vi "SMTP Email Send Message End.vi"(4 "error in (no error)":errorcluster caption="entrée d'erreur (pas d'erreur)", 7 "smtp session":T1 caption="session smtp") -> (0 "error out":errorcluster caption="sortie d'erreur", 1 "reply":string caption="réponse", 2 "reply code":i32 caption="code de réponse", 3 "smtp session out":T1 caption="session smtp en sortie")   [LabVIEW 2022 SP3, in "Copie de NI_SMTPEmail.lvlib"]
doc: "Envoie un commande de fin de données ('end of DATA') à un serveur SMTP à travers la connexion TCP décrite par \"Session SMTP\", reçoit la réponse et l'interprète. Le VI renvoie une \"session SMTP en sortie\" et les résultats d'interprétation de l'erreur dans le cluster de sortie d'erreur."
uses:
  Copie de NI_SMTPEmail.lvlib
  SMTP Email Session.ctl
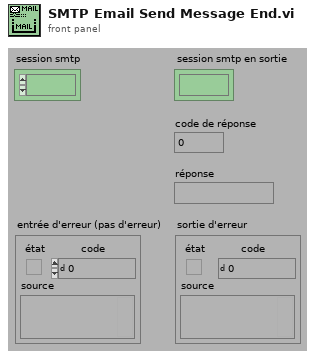
[diagram p1: front panel]
types:
  T1 = typedef "Copie de NI_SMTPEmail.lvlib/SMTP Email Session.ctl" = refnum<k1>
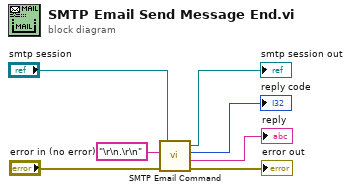
[diagram p0: block diagram]
diagram:
  n1 = call "SMTP Email Command.vi"("error in (no error)"="error in (no error)", "command"="\r\n.\r\n", "smtp session"="smtp session") -> ("error out"=→"error out":errorcluster, "reply"=→"reply":string, "reply code"=→"reply code":i32, "smtp session out"=→"smtp session out":T1)  [unwired: 1 in]
